vi "C_HDLC_State_Init.vi"(8 "error in (no error)":errorcluster) -> (0 "error out":errorcluster, 3 "C_State":T1)   [LabVIEW 2021, in "CANsub_C.lvlib"]
doc: "Creates a new HDLC decoder state (4112 bytes) for C_HDLC_Decode. Use one state per byte stream and keep it in a shift register."
uses:
  CANsub_C.lvlib
  codec_vis/CANsub_Codec.lvlib
  C_State.ctl
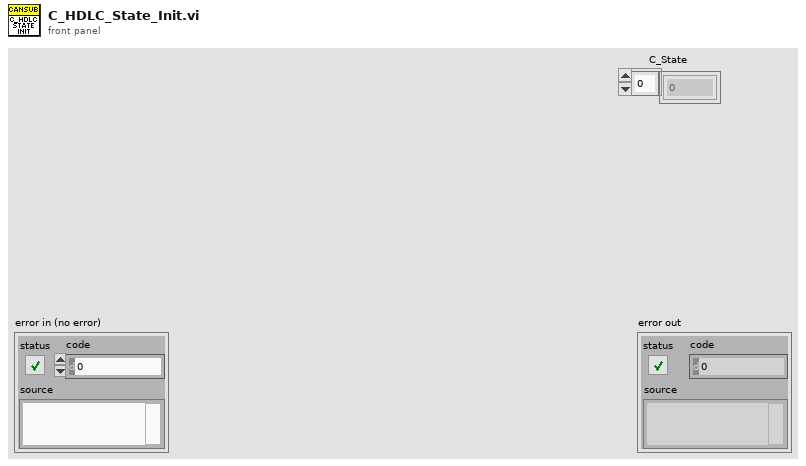
[diagram p1: front panel]
types:
  T1 = typedef "CANsub_C.lvlib/C_State.ctl" = u8[]
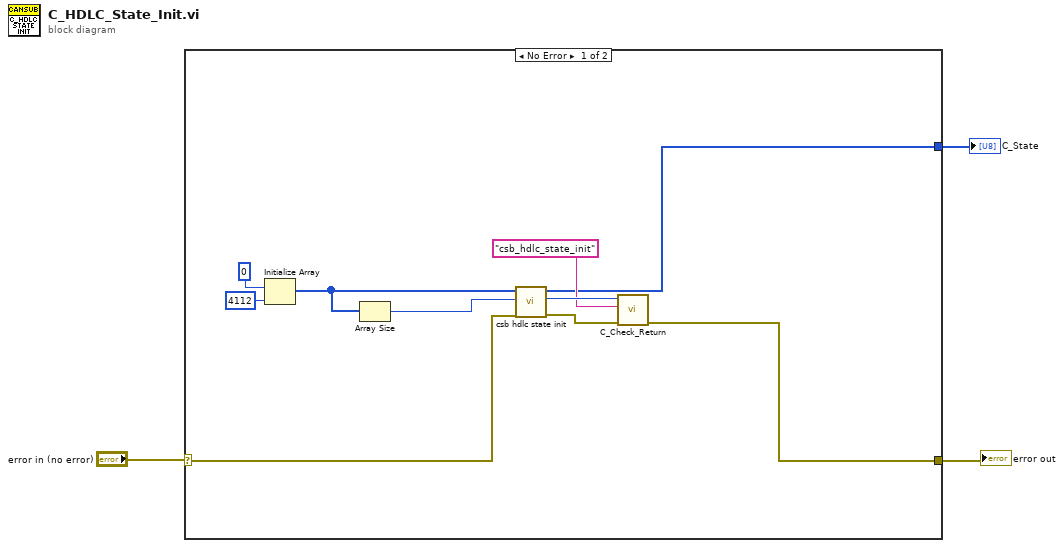
[diagram p0: block diagram]
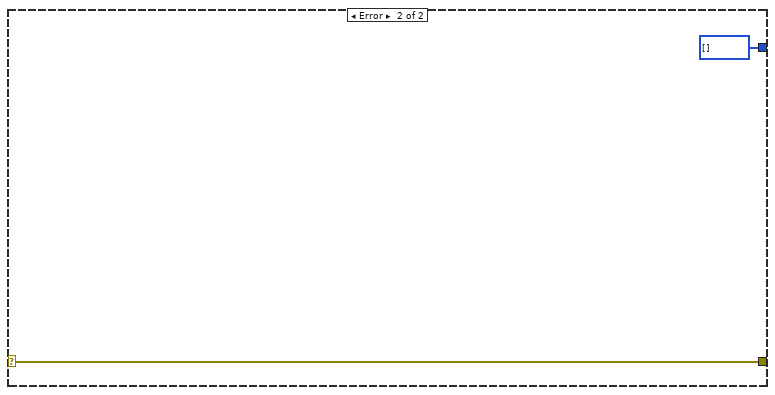
[diagram p2: hidden frame]
diagram:
  n1 = case shown="No Error" "error in (no error)" {
    selector: "error in (no error)" -> [w9 w15]
    tunnel: [w4 w15] -> w2
    tunnel: [w6 u8[] [] ("state out")] -> w1
    frame No Error {
      n2 = Initialize Array(u8 0, 4112 ("dimension size")) -> (w11:u8[])
      n3 = Array Size(array=w11) -> (size(s)=w10:i32)
      n4 = call "csb hdlc state init.vi"("error in (no error)"=w9, "state_size"=w10, "state"=w11) -> ("error out"=w5:errorcluster, "function return"=w8:i32, "state out"=w6:u8[])  [unwired: 6 in]
      n5 = call "C_Check_Return.vi"("error in (no error)"=w5, "function name"="csb_hdlc_state_init", "function return"=w8) -> ("error out"=w4:errorcluster)  [unwired: 6 in, 2 out]
    }
    frame Error {
    }
  }
  "error out" <- w2
  "C_State" <- w1
